vi "Update Basic Components.vi"(8 "error in (no error)":errorcluster, 11 "HistorianCharting in":refnum<class "HistorianCharting.lvclass">) -> (0 "error out":errorcluster, 3 "HistorianCharting out":refnum<class "HistorianCharting.lvclass">)   [LabVIEW 2020, in "VolatusGUIElements.lvlib" / "HistorianCharting.lvclass"]
uses:
  HistorianCharting.lvclass
  HistorianCharting.lvclass/HistorianCharting.ctl
  <vilib>/dlg_ctls.llb/Space Constant.vi
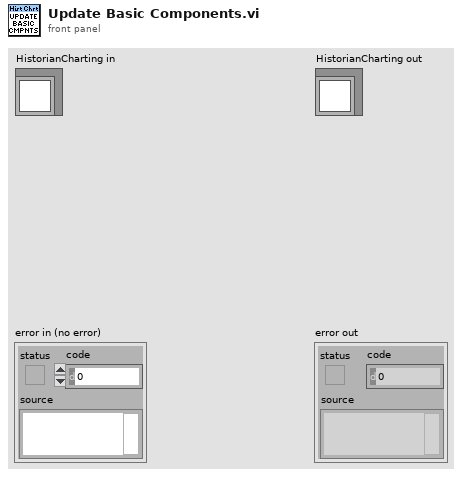
[diagram p1: front panel]
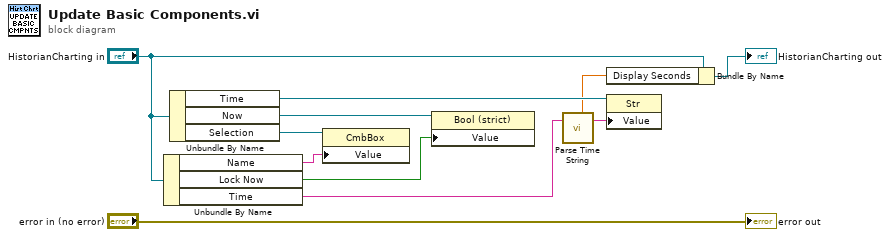
[diagram p0: block diagram]
diagram:
  n1 = Unbundle By Name("HistorianCharting in") -> ("Name"=w8:string, "Lock Now"=w6:bool, "Time"=w4:string)
  n2 = Unbundle By Name("HistorianCharting in") -> ("Time"=w5:refnum<vi>, "Now"=w7:refnum<vi>, "Selection"=w9:refnum<vi>)
  n3 = property class="CmbBox"(reference=w9, "Value"=w8) -> ()  [unwired: 1 in, 2 out]
  n4 = property class="Bool (strict)"(reference=w7, "Value"=w6) -> ()  [unwired: 1 in, 2 out]
  n5 = call "Parse Time String.vi"("Time String"=w4) -> ("Seconds"=w1:dbl, "Normalized String"=w3:string)  [unwired: 5 in]
  n6 = Bundle By Name(cluster="HistorianCharting in", "Display Seconds"=w1) -> (→"HistorianCharting out":refnum<class "HistorianCharting.lvclass">)
  n7 = property class="Str"(reference=w5, "Value"=w3) -> ()  [unwired: 1 in, 2 out]
  "error out" <- "error in (no error)"
